vi "RDC-Array-calc_cf_c0_m1.vi"(10 "water":T1, 11 "Open":T1) -> (2 "C0":dbl[](array[numeric]), 3 "cf":dbl[](array[numeric]))   [LabVIEW 2020, in "RDC-Reflection_Data_Computation.lvlib"]
doc: "Computes the C0 and cf arrays per frequency from a water and an Open Common Format cluster."
uses:
  RDC-Reflection_Data_Computation.lvlib
  Reflector/RFH-common_data_format.ctl
  Reflector/RFH-Reflection_File_Handler.lvlib
panel:
  out "Er*c0  + cf g":cluster{"Frequency":dbl[], dbl[]}(graph)
  out "Ctot":cluster{"Frequency":dbl[], dbl[]}(graph)
  out "Cf":cluster{"Frequency":dbl[], dbl[]}(graph)
  out "Er*c0  + cf":dbl[](array[numeric])
  out "C0 g":cluster{"Frequency":dbl[], dbl[]}(graph)
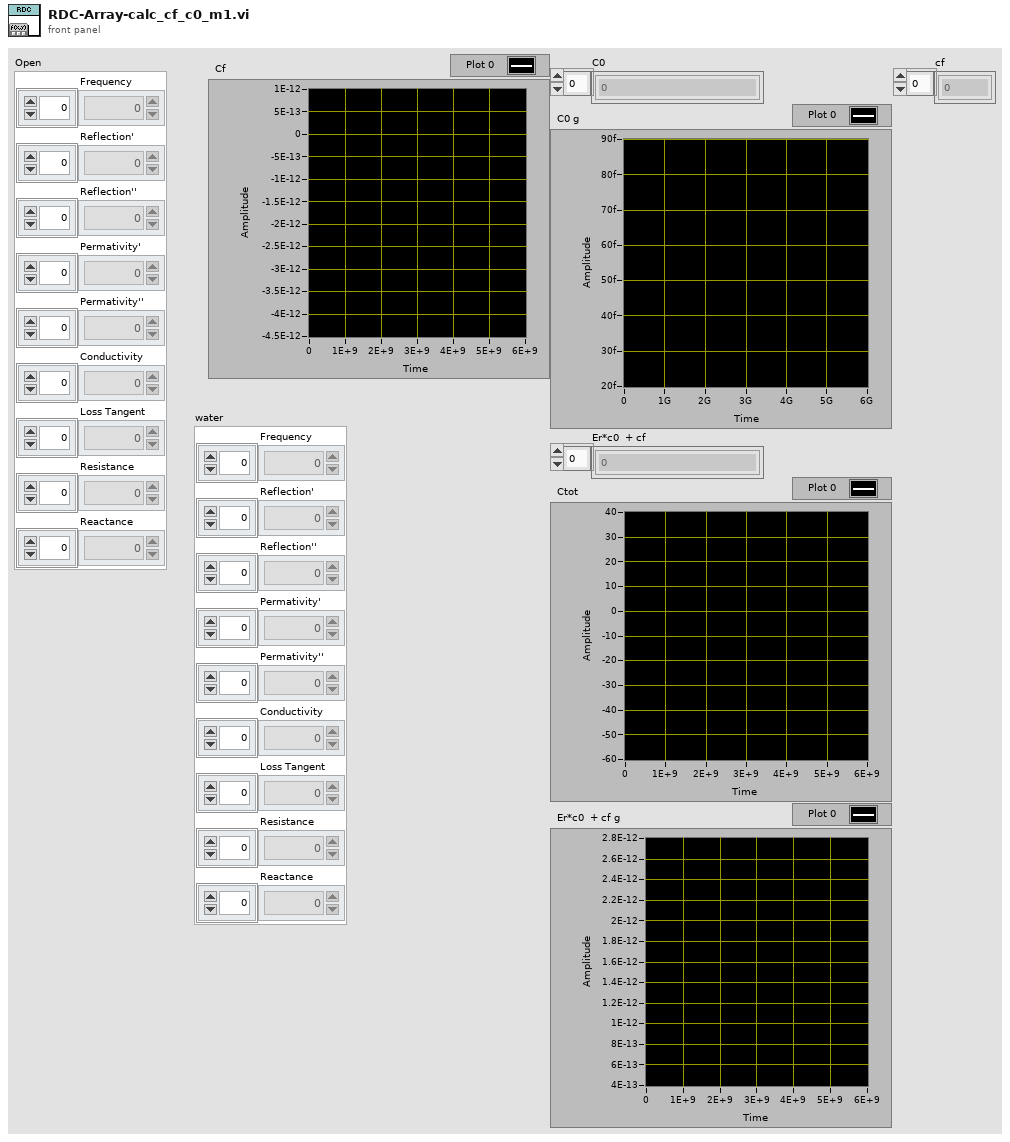
[diagram p1: front panel]
types:
  T1 = typedef "RFH-Reflection_File_Handler.lvlib/RFH-common_data_format.ctl" = cluster{"Frequency":dbl[], "Reflection'":dbl[], "Reflection''":dbl[], "Permativity'":dbl[], "Permativity''":dbl[], "Conductivity":dbl[], "Loss Tangent":dbl[], "Resistance":dbl[], "Reactance":dbl[]}
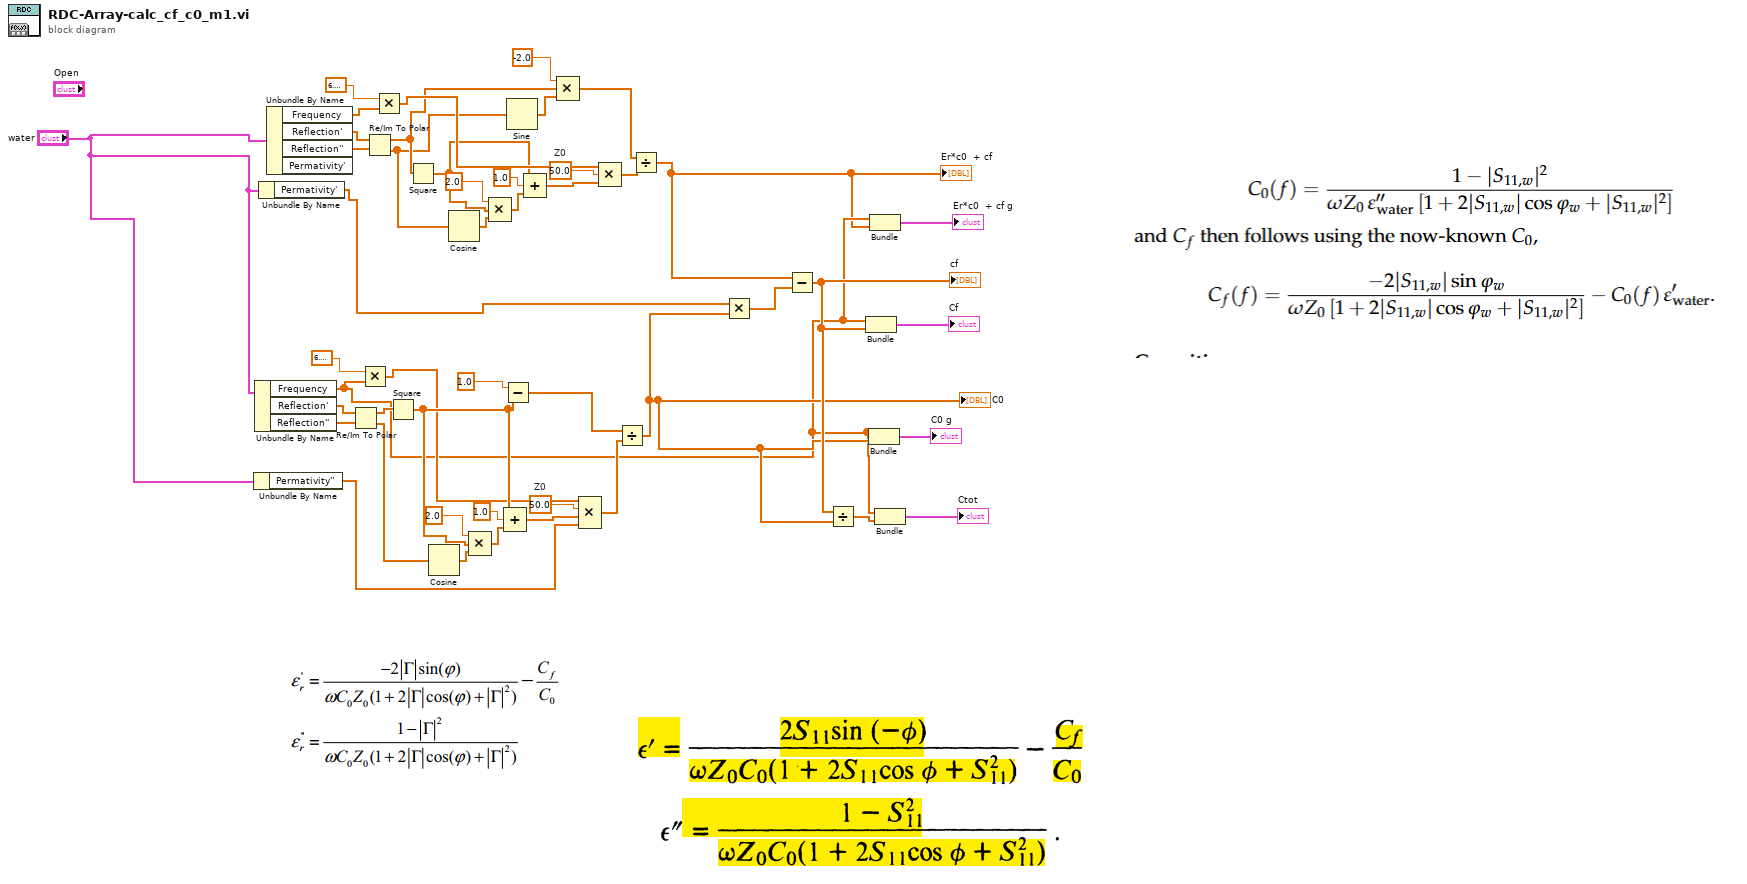
[diagram p0: block diagram]
diagram:
  w26 = 50.0  # Z0
  w35 = 50.0  # Z0
  n1 = Unbundle By Name("water") -> ("Permativity''"=w2:dbl[])
  n2 = Unbundle By Name("water") -> ("Frequency"=w5:dbl[], "Reflection'"=w47:dbl[], "Reflection''"=w46:dbl[])
  n3 = Unbundle By Name("water") -> ("Permativity'"=w3:dbl[])
  n4 = Unbundle By Name("water") -> ("Frequency"=w30:dbl[], "Reflection'"=w18:dbl[], "Reflection''"=w19:dbl[])  [unwired: 1 out]
  n5 = Re/Im To Polar(2:w46, 3:w47) -> (0:w41:dbl[], 1:w45:dbl[])
  n6 = Multiply(x=6.283185307179586, y=w5) -> (x*y=w32:dbl[])
  n7 = Re/Im To Polar(2:w19, 3:w18) -> (0:w15:dbl[], 1:w16:dbl[])
  n8 = Multiply(x=6.283185307179586, y=w30) -> (x*y=w29:dbl[])
  n9 = Square(x=w45) -> (x^2=w39:dbl[])
  n10 = Square(x=w16) -> (x^2=w22:dbl[])
  n11 = Cosine(x=w41) -> (cos(x)=w40:dbl[])
  n12 = Cosine(x=w15) -> (cos(x)=w21:dbl[])
  n13 = Compound Arithmetic op=MULTIPLY(2.0, w39, w40) -> (w37:dbl[])
  n14 = Compound Arithmetic op=MULTIPLY(2.0, w22, w21) -> (w24:dbl[])
  n15 = Subtract(x=1.0, y=w39) -> (x-y=w43:dbl[])
  n16 = Compound Arithmetic op=ADD(w39, 1.0, w37) -> (w36:dbl[])
  n17 = Sine(x=w15) -> (sin(x)=w14:dbl[])
  n18 = Compound Arithmetic op=ADD(w22, 1.0, w24) -> (w25:dbl[])
  n19 = Compound Arithmetic op=MULTIPLY(-2.0, w16, w14) -> (w13:dbl[])
  n20 = Compound Arithmetic op=MULTIPLY(w32, w35, w36, w2) -> (w33:dbl[])
  n21 = Compound Arithmetic op=MULTIPLY(w29, w26, w25) -> (w28:dbl[])
  n22 = Divide(x=w43, y=w33) -> (x/y=w8:dbl[])
  "C0" <- w8
  n23 = Divide(x=w13, y=w28) -> (x/y=w4:dbl[])
  "Er*c0  + cf" <- w4
  n24 = Multiply(x=w3, y=w8) -> (x*y=w11:dbl[])
  n25 = Subtract(x=w4, y=w11) -> (x-y=w9:dbl[])
  "cf" <- w9
  n26 = Divide(x=w9, y=w8) -> (x/y=w7:dbl[])
  n27 = Bundle("Frequency"=w5, w9) -> (→"Cf":cluster{"Frequency":dbl[], dbl[]})  [unwired: 1 in]
  n28 = Bundle("Frequency"=w5, w8) -> (→"C0 g":cluster{"Frequency":dbl[], dbl[]})  [unwired: 1 in]
  n29 = Bundle("Frequency"=w5, w4) -> (→"Er*c0  + cf g":cluster{"Frequency":dbl[], dbl[]})  [unwired: 1 in]
  n30 = Bundle("Frequency"=w5, w7) -> (→"Ctot":cluster{"Frequency":dbl[], dbl[]})  [unwired: 1 in]
